vi "VIrefDB.vi"(11 "spawned VI ref":refnum<vi>) -> (3 "spawned VI refs":refnum<vi>[](array[refnum]))   [LabVIEW 2023, in "GettingStartedWindow.lvlib"]
uses:
  <resource>/modes/FRC/GettingStartedWindow.lvlib
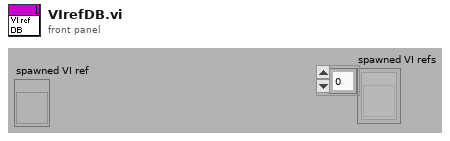
[diagram p1: front panel]
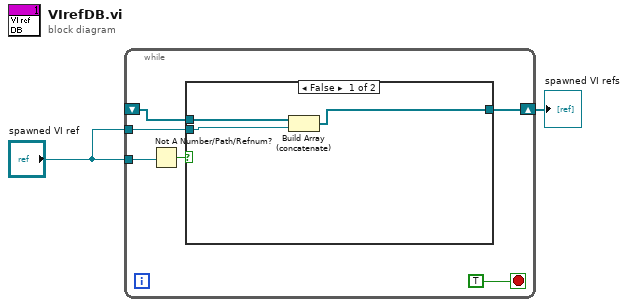
[diagram p0: block diagram]
diagram:
  n1 = while {
    shift-right: [w5] -> w1
    shift-left: _ -> [w4]
    tunnel: "spawned VI ref" -> [w7]
    tunnel: "spawned VI ref" -> [w3]
    stop <- TRUE stop-if-true
    n2 = Not A Number/Path/Refnum?(number/path/refnum=w7) -> (NaN/Path/Refnum?=w6:bool)
    n3 = case shown="False" w6 {
      tunnel: [w11 w12] -> w5
      tunnel: w4 -> [w10 w12]
      tunnel: w3 -> [w9 _]
      frame False {
        n4 = Build Array (concatenate)(w10, w9) -> (w11:refnum<vi>[])
      }
      frame True {
      }
    }
  }
  "spawned VI refs" <- w1
